vi "Validate Password.vi"(4 "error in (no error)":errorcluster, 5 "Password":string, 6 "LoginName":string, 7 "EasyUserManager in":refnum<class "EasyUserManager.lvclass">) -> (0 "error out":errorcluster, 2 "Password OK":bool, 3 "EasyUserManager out":refnum<class "EasyUserManager.lvclass">)   [LabVIEW 2024, in "EasyUserManager.lvclass"]
doc: "Validate the provided <B>Password</B> for the user specified by <B>LoginName</B>."
uses:
  EasyUserManager.lvclass
  EasyUserManager.lvclass/EasyUserManager.ctl
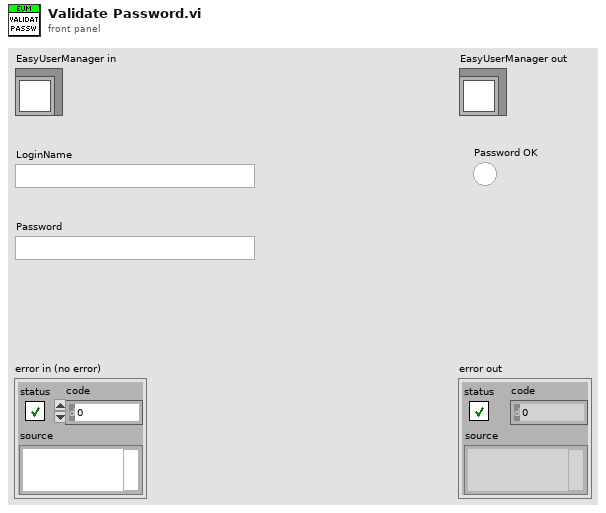
[diagram p1: front panel]
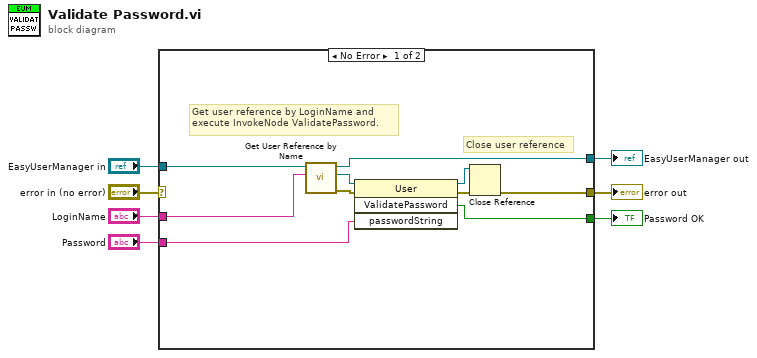
[diagram p0: block diagram]
diagram:
  n1 = case shown="No Error" "error in (no error)" {
    selector: "error in (no error)" -> [_ w19]
    tunnel: [w15 w19] -> w6
    tunnel: [w17 w18] -> w4
    tunnel: "EasyUserManager in" -> [w16 w18]
    tunnel: "LoginName" -> [w10 _]
    tunnel: "Password" -> [w9 _]
    tunnel: [w8 _] -> w1
    frame No Error {
      # "Close user reference"
      # "Get user reference by LoginName and\nexecute InvokeNode ValidatePassword."
      n2 = call "Get User Reference by Name.vi"("LoginName"=w10, "EasyUserManager in"=w16) -> ("error out"=w12:errorcluster, "User Reference"=w14:refnum<k7>, "EasyUserManager out"=w17:refnum<class "EasyUserManager.lvclass">)  [unwired: 3 in]
      n3 = invoke on="Invoke Node" class="User" method="ValidatePassword"(reference=w14, error in=w12, "passwordString"=w9) -> (reference out=w11:refnum<k7>, error out=w13:errorcluster, "ValidatePassword"=w8:bool)  [unwired: 1 in, 1 out]
      n4 = Close Reference(reference=w11, error in (no error)=w13) -> (error out=w15:errorcluster)
    }
    frame Error {
      # "Pass error and do nothing."
    }
  }
  "error out" <- w6
  "EasyUserManager out" <- w4
  "Password OK" <- w1
